vi "measure CE OOB per BW With Stop Enable.vi"(8 "error in (no error)":errorcluster, 10 "Ref - Test Stop Button":refnum<vi>, 11 "SA Measurement in":refnum<class "SA Measurement.lvclass">) -> (0 "error out":errorcluster, 2 "Marker Amplitude":dbl, 3 "SA Measurement out":refnum<class "SA Measurement.lvclass">)   [LabVIEW 2023, in "Spectrum Analyzer.lvlib" / "SA Measurement.lvclass"]
uses:
  SA Measurement.lvclass
  SA Measurement.lvclass/SA Measurement.ctl
  TYPE DEFINITION/TYPE RBW and VBW Select.ctl
  Spectrum Analyzer.lvlib
  TYPE DEFINITION/TYPE Marker Peak Search Type.ctl
  Interface_Spectrum/Interface_Spectrum.lvclass
  TYPE DEFINITION/Keysight 9020A/TYPE Measurement Preset.ctl
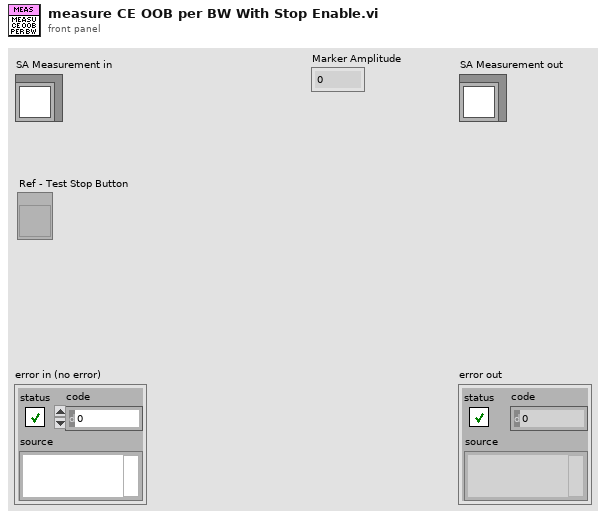
[diagram p1: front panel]
types:
  T1 = enum16{"Free Run", "Video (IF Envelop)", "RF Burst"}
  T2 = typedef "Spectrum Analyzer.lvlib/TYPE Measurement Preset.ctl" = enum16{"Sweep SA Mode", "Channel Power", "Occupied BW", "ACP", "Spurious Emission", "Spurious Emission Mask", "Burst Power (Transmit Power)"}
  T3 = typedef "Spectrum Analyzer.lvlib/TYPE Marker Peak Search Type.ctl" = enum16{"Max", "Next Peak"}
  T4 = typedef "Spectrum Analyzer.lvlib/TYPE RBW and VBW Select.ctl" = enum16{"Res BW", "Video BW"}
  T5 = typedef "Spectrum Analyzer.lvlib/TYPE Y-axis Unit.ctl" = enum16{"dBm", "dBmV", "dBuV", "dBpW", "Volt", "Ampere", "Watt"}
  T6 = typedef "Spectrum Analyzer.lvlib/TYPE Display Trace Mode Select.ctl" = enum16{"Clear Write", "Max Hold", "Min Hold", "Average", "View"}
  T7 = typedef "Spectrum Analyzer.lvlib/TYPE Detect Mode Select.ctl" = enum16{"Det Auto (Normal)", "Auto Peak", "Positive Peak", "Negative Peak", "Sample", "RMS", "Average", "Quasipeak", "CISPR Average", "RMS Average"}
  T8 = cluster{"Trace Mode":T6, "Detector Type":T7, "Detect Auto?":bool}[]
  T9 = typedef "Spectrum Analyzer.lvlib/TYPE Marker Value.ctl" = cluster{"X-axis":dbl, "Y-axis":dbl}
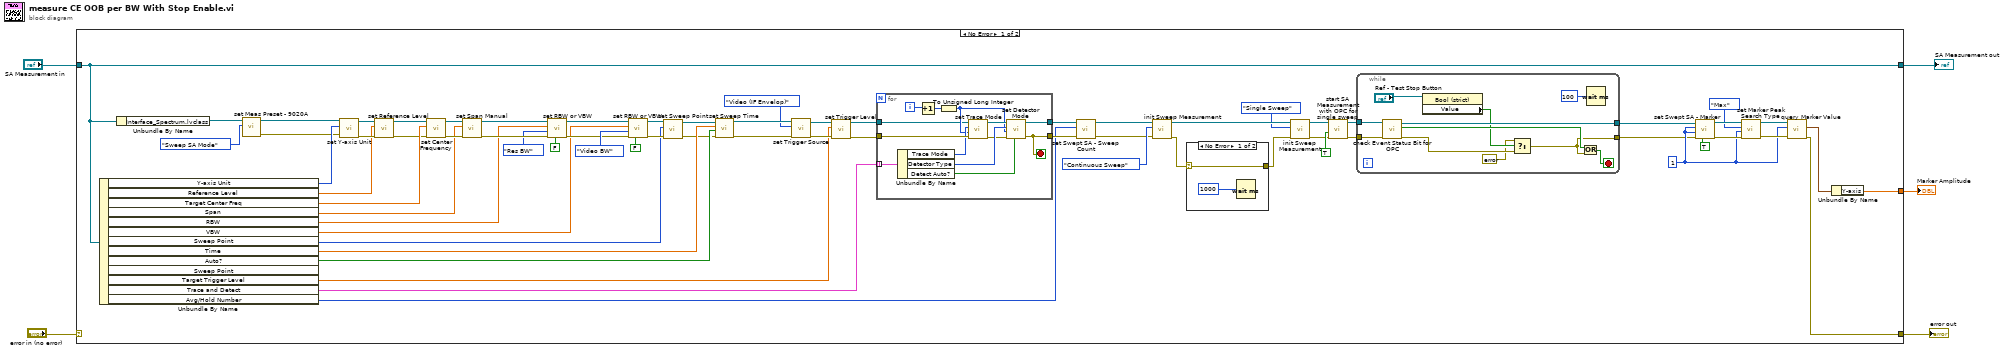
[diagram p0: block diagram]
diagram:
  n1 = case shown="No Error" "error in (no error)" {
    selector: "error in (no error)" -> [_ w102]
    tunnel: [w23 w102] -> w2
    tunnel: [w24 w101] -> w3
    tunnel: "SA Measurement in" -> [w24 w101]
    tunnel: [w22 _] -> w1
    frame No Error {
      w47 = 1 ("Index")
      n2 = Unbundle By Name(w24) -> ("Y-axis Unit"=w59:T5, "Reference Level"=w44:dbl, "Target Center Freq"=w73:dbl, "Span"=w70:dbl, "RBW"=w67:dbl, "VBW"=w60:dbl, "Sweep Point"=w16:u32, "Time"=w58:dbl, "Auto?"=w57:bool, "Target Trigger Level"=w6:dbl, "Trace and Detect"=w56:T8, "Avg/Hold Number"=w30:u32)  [unwired: 1 out]
      n3 = Unbundle By Name(w24) -> ("Interface_Spectrum.lvclass"=w40:refnum<class "Interface_Spectrum.lvclass">)
      n4 = call-dynamic "set Meas Preset - 9020A.vi"("Measurement Preset"=TYPE_Measurement_Preset."Sweep SA Mode", "Interface_Spectrum in"=w40) -> ("error out"=w38:errorcluster, "Interface_Spectrum out"=w39:refnum<class "Interface_Spectrum.lvclass">)  [unwired: 8 in]
      n5 = call-dynamic "set Y-axis Unit.vi"("error in (no error)"=w38, "Y-axis Unit"=w59, "Interface_Spectrum in"=w39) -> ("error out"=w45:errorcluster, "Interface_Spectrum out"=w46:refnum<class "Interface_Spectrum.lvclass">)  [unwired: 7 in]
      n6 = call-dynamic "set Reference Level.vi"("error in (no error)"=w45, "Reference Level"=w44, "Interface_Spectrum in"=w46) -> ("error out"=w42:errorcluster, "Interface_Spectrum out"=w43:refnum<class "Interface_Spectrum.lvclass">)  [unwired: 7 in]
      n7 = call-dynamic "set Center Frequency.vi"("error in (no error)"=w42, "Center Frequency (Hz)"=w73, "Interface_Spectrum in"=w43) -> ("error out"=w71:errorcluster, "Interface_Spectrum out"=w72:refnum<class "Interface_Spectrum.lvclass">)  [unwired: 7 in]
      n8 = call-dynamic "set Span Manual.vi"("error in (no error)"=w71, "Span (Hz)"=w70, "Interface_Spectrum in"=w72) -> ("error out"=w68:errorcluster, "Interface_Spectrum out"=w69:refnum<class "Interface_Spectrum.lvclass">)  [unwired: 7 in]
      n9 = call-dynamic "set RBW or VBW.vi"("BW Auto?"=FALSE, "error in (no error)"=w68, "BW Type"=TYPE_RBW_and_VBW_Select."Res BW", "BW Value (Hz)"=w67, "Interface_Spectrum in"=w69) -> ("error out"=w61:errorcluster, "Interface_Spectrum out"=w62:refnum<class "Interface_Spectrum.lvclass">)  [unwired: 5 in]
      n10 = call-dynamic "set RBW or VBW.vi"("BW Auto?"=FALSE, "error in (no error)"=w61, "BW Type"=TYPE_RBW_and_VBW_Select."Video BW", "BW Value (Hz)"=w60, "Interface_Spectrum in"=w62) -> ("error out"=w18:errorcluster, "Interface_Spectrum out"=w17:refnum<class "Interface_Spectrum.lvclass">)  [unwired: 5 in]
      n11 = call-dynamic "set Sweep Point.vi"("error in (no error)"=w18, "Sweep Point"=w16, "Interface_Spectrum in"=w17) -> ("error out"=w14:errorcluster, "Interface_Spectrum out"=w15:refnum<class "Interface_Spectrum.lvclass">)  [unwired: 7 in]
      n12 = call-dynamic "set Sweep Time.vi"("error in (no error)"=w14, "Sweep Time Auto?"=w57, "Sweep Time(sec)"=w58, "Interface_Spectrum in"=w15) -> ("error out"=w35:errorcluster, "Interface_Spectrum out"=w36:refnum<class "Interface_Spectrum.lvclass">)  [unwired: 6 in]
      n13 = call-dynamic "set Trigger Source.vi"("error in (no error)"=w35, "Trigger Source"=T1."Video (IF Envelop)", "Interface_Spectrum in"=w36) -> ("error out"=w32:errorcluster, "Interface_Spectrum out"=w33:refnum<class "Interface_Spectrum.lvclass">)  [unwired: 7 in]
      n14 = call-dynamic "set Trigger Level.vi"("error in (no error)"=w32, "Trigger Level (dBm)"=w6, "Interface_Spectrum in"=w33) -> ("error out"=w31:errorcluster, "Interface_Spectrum out"=w29:refnum<class "Interface_Spectrum.lvclass">)  [unwired: 7 in]
      n15 = for {
        tunnel: w31 -> [w99]
        tunnel: w56 -> [w100] mode=indexing
        tunnel: [w89] -> w54
        tunnel: [w90] -> w55
        tunnel: w29 -> [w88]
        i -> [w98]
        stop <- w89 stop-if-true
        n16 = Unbundle By Name(w100) -> ("Trace Mode"=w96:T6, "Detector Type"=w94:T7, "Detect Auto?"=w91:bool)
        n17 = Increment(x=w98) -> (x+1=w97:i32)
        n18 = To Unsigned Long Integer(number=w97) -> (unsigned 32bit integer=w92:u32)
        n19 = call-dynamic "set Trace Mode.vi"("error in (no error)"=w99, "Trace Index"=w92, "Trace Mode"=w96, "Interface_Spectrum in"=w88) -> ("error out"=w93:errorcluster, "Interface_Spectrum out"=w95:refnum<class "Interface_Spectrum.lvclass">)  [unwired: 6 in]
        n20 = call-dynamic "set Detector Mode.vi"("Detect Auto?"=w91, "error in (no error)"=w93, "Trace Index"=w92, "Detector Type"=w94, "Interface_Spectrum in"=w95) -> ("error out"=w89:errorcluster, "Interface_Spectrum out"=w90:refnum<class "Interface_Spectrum.lvclass">)  [unwired: 5 in]
      }
      n21 = call-dynamic "set Swept SA - Sweep Count.vi"("error in (no error)"=w54, "Sweep Count"=w30, "Interface_Spectrum in"=w55) -> ("error out"=w26:errorcluster, "Interface_Spectrum out"=w27:refnum<class "Interface_Spectrum.lvclass">)  [unwired: 7 in]
      n22 = call-dynamic "init Sweep Measurement.vi"("error in (no error)"=w26, "Sweep Measurement Mode"=enum16{"Single Sweep", "Continuous Sweep"}."Continuous Sweep", "Interface_Spectrum in"=w27) -> ("error out"=w25:errorcluster, "Interface_Spectrum out"=w21:refnum<class "Interface_Spectrum.lvclass">)  [unwired: 7 in]
      n23 = case shown="No Error" w25 {
        selector: w25 -> [w85 w87]
        tunnel: [w85 w87] -> w20
        frame No Error {
          n24 = Wait (ms)(milliseconds to wait=u32 1000) -> ()  [unwired: 1 out]
        }
        frame Error {
        }
      }
      n25 = call-dynamic "init Sweep Measurement.vi"("error in (no error)"=w20, "Sweep Measurement Mode"=enum16{"Single Sweep", "Continuous Sweep"}."Single Sweep", "Interface_Spectrum in"=w21) -> ("error out"=w9:errorcluster, "Interface_Spectrum out"=w10:refnum<class "Interface_Spectrum.lvclass">)  [unwired: 7 in]
      n26 = call-dynamic "start SA Measurement with OPC for single sweep.vi"("error in (no error)"=w9, "with OPC?"=TRUE, "Interface_Spectrum in"=w10) -> ("error out"=w11:errorcluster, "Interface_Spectrum out"=w12:refnum<class "Interface_Spectrum.lvclass">)  [unwired: 7 in]
      n27 = while {
        tunnel: w12 -> [w84]
        tunnel: w11 -> [w83]
        tunnel: [w74] -> w7
        tunnel: [w80] -> w8
        stop <- w81 stop-if-true
        n28 = call-dynamic "check Event Status Bit for OPC.vi"("error in (no error)"=w83, "Interface_Spectrum in"=w84) -> ("error out"=w76:errorcluster, "OPC Bit Changed?"=w82:bool, "Interface_Spectrum out"=w80:refnum<class "Interface_Spectrum.lvclass">)  [unwired: 7 in]
        n29 = property class="Bool (strict)"(reference="Ref - Test Stop Button") -> ("Value"=w77:bool)  [unwired: 1 in, 2 out]
        n30 = Select(t=errorcluster {"status"=TRUE, "code"=0, "source"=""}, s=w77, f=w76) -> (s? t:f=w74:errorcluster)
        n31 = Or(x=w82, y=w74) -> (x .or. y?=w81:bool)
        n32 = Wait (ms)(milliseconds to wait=u32 100) -> ()  [unwired: 1 out]
      }
      n33 = call-dynamic "set Swept SA - Marker.vi"("On?"=TRUE, "error in (no error)"=w7, "trace"=w47, "Index"=w47, "Interface_Spectrum in"=w8) -> ("error out"=w51:errorcluster, "Interface_Spectrum out"=w52:refnum<class "Interface_Spectrum.lvclass">)  [unwired: 5 in]
      n34 = call-dynamic "set Marker Peak Search Type.vi"("error in (no error)"=w51, "Marker Index"=w47, "Peak Search Type"=TYPE_Marker_Peak_Search_Type."Max", "Interface_Spectrum in"=w52) -> ("error out"=w48:errorcluster, "Interface_Spectrum out"=w49:refnum<class "Interface_Spectrum.lvclass">)  [unwired: 6 in]
      n35 = call-dynamic "query Marker Value.vi"("error in (no error)"=w48, "Marker Index"=w47, "Interface_Spectrum in"=w49) -> ("error out"=w23:errorcluster, "Marker Value"=w41:T9)  [unwired: 6 in, 1 out]
      n36 = Unbundle By Name(w41) -> ("Y-axis"=w22:dbl)
    }
    frame Error {
    }
  }
  "error out" <- w2
  "SA Measurement out" <- w3
  "Marker Amplitude" <- w1
